vi "Connect-Disconnect.vi"(7 "Address":string, 8 "Error In":errorcluster) -> (0 "Error Out":errorcluster)   [LabVIEW 2018, in "Tests.lvlib" / "Session.lvlib"]
uses:
  Session.lvlib
  src/Toolkit/Session/Support/Create from SSH.vi
  src/Toolkit/Session/Support/Destroy to SSH.vi
  <vilib>/addons/_JKI Toolkits/Caraya/classes/Test/Test.lvclass
  src/Toolkit/SSH/SSH.lvclass
  src/Toolkit/Session/Session.lvclass
  <vilib>/addons/_JKI Toolkits/Caraya/classes/Assert/Assert.lvclass
  Tests.lvlib
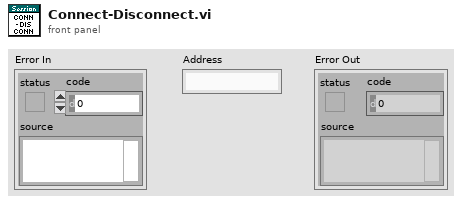
[diagram p1: front panel]
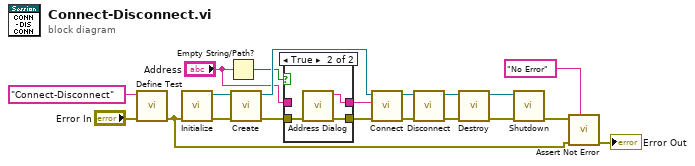
[diagram p0: block diagram]
diagram:
  n1 = call <vilib>:"Define Test.vi"("error in (no error)"="Error In", "Label (VI Title)"="Connect-Disconnect") -> ("error out"=w13:errorcluster)  [unwired: 9 in]
  n2 = call "Initialize.vi"("Error In"=w13) -> ("Error Out"=w18:errorcluster, "SSH"=w17:refnum<class "SSH.lvclass">)  [unwired: 9 in]
  n3 = Empty String/Path?(string/path="Address") -> (empty?=w7:bool)
  n4 = call-poly "Create.vi"("Error In"=w18, "SSH"=w17) -> ("Error Out"=w4:errorcluster, "Sesssion"=w11:refnum<class "Session.lvclass">)  [unwired: 8 in]
  n5 = case shown="True" w7 {
    tunnel: w4 -> [w21 w25]
    tunnel: [w21 w24] -> w5
    tunnel: [w22 w23] -> w6
    tunnel: "Address" -> [w22 _]
    frame False {
    }
    frame True {
      n6 = call "Address Dialog.vi"("Error In"=w25) -> ("Error Out"=w24:errorcluster, "Address Out"=w23:string)  [unwired: 9 in]
    }
  }
  n7 = call "Connect.vi"("Error In"=w5, "Address"=w6, "Session In"=w11) -> ("Error Out"=w8:errorcluster, "Sesssion Out"=w9:refnum<class "Session.lvclass">)  [unwired: 7 in]
  n8 = call "Disconnect.vi"("Error In"=w8, "Session In"=w9) -> ("Error Out"=w1:errorcluster, "Sesssion Out"=w10:refnum<class "Session.lvclass">)  [unwired: 8 in]
  n9 = call-poly "Destroy.vi"("Error In"=w1, "Session"=w10) -> ("Error Out"=w2:errorcluster, "SSH"=w16:refnum<class "SSH.lvclass">)  [unwired: 8 in]
  n10 = call "Shutdown.vi"("Error In"=w2, "SSH"=w16) -> ("Error Out"=w15:errorcluster)  [unwired: 9 in]
  n11 = call <vilib>:"Assert Not Error.vi"("Label"="No Error", "error in (no error)"=w13, "Not Error?"=w15) -> ("error out"=→"Error Out":errorcluster)  [unwired: 8 in]
